vi "Pi_Test.vi"() -> ()   [LabVIEW 2024]
panel:
  out "Current MW Value":dbl
  out "Waveform Chart":dbl[](graph)
  out "output array":dbl[](array[numeric])
  in  "Pi/2 time":dbl=2e-09
  in  "N per point":i32
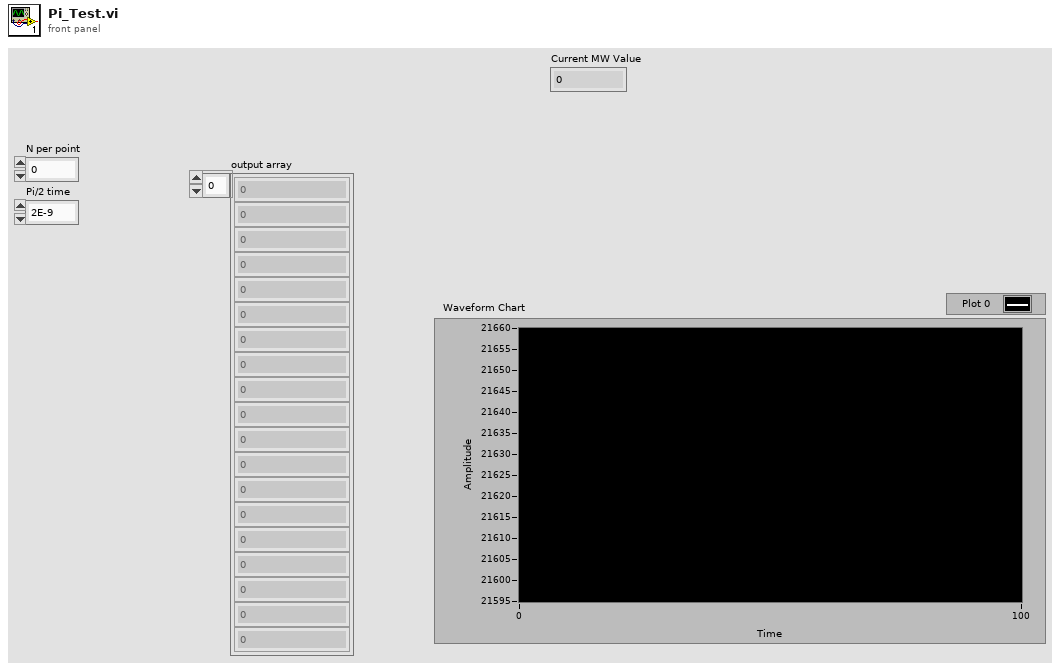
[diagram p1: front panel]
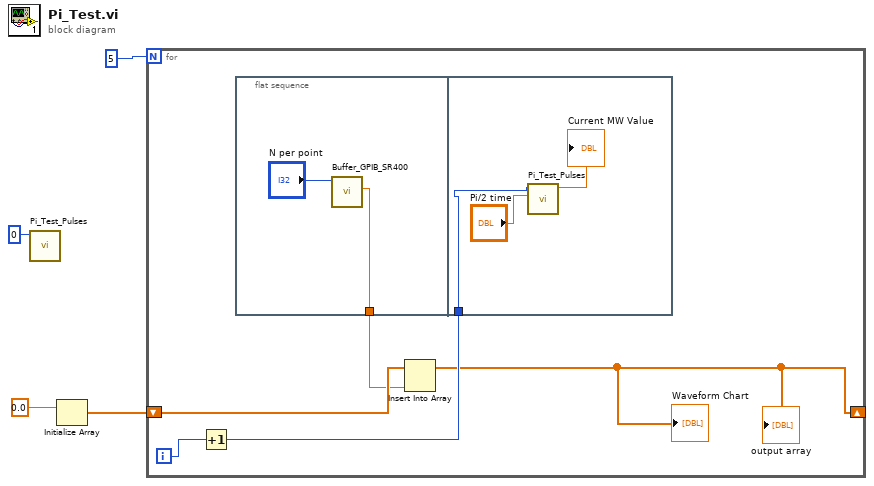
[diagram p0: block diagram]
diagram:
  n1 = call "Pi_Test_Pulses.vi"("Numeric"=0) -> ()  [unwired: 10 in, 1 out]
  n2 = Initialize Array(0.0) -> (w3:dbl[])  [unwired: 1 in]
  n3 = for {
    N: 5 -> [_]
    shift-right: [w5] -> _
    shift-left: w3 -> [w7]
    i -> [w9]
    n4 = Increment(x=w9) -> (x+1=w8:i32)
    n5 = flat-sequence {
      tunnel: [w10] -> w6
      tunnel: w8 -> [w13]
      frame #0 {
        n6 = call "Buffer_GPIB_SR400.vi"("N per point"="N per point") -> ("x/y"=w10:dbl)  [unwired: 9 in, 1 out]
      }
      frame #1 {
        n7 = call "Pi_Test_Pulses.vi"("Pi/2 time"="Pi/2 time", "Numeric"=w13) -> ("x+y"=→"Current MW Value":dbl)  [unwired: 9 in]
      }
    }
    n8 = Insert Into Array(array=w7, new element=w6) -> (w5:dbl[])  [unwired: 1 in]
    "output array" <- w5
    "Waveform Chart" <- w5
  }
